vi "libssh2_userauth_authenticated.vi"(8 "error in (no error)":errorcluster, 11 "session":T1) -> (0 "error out":errorcluster, 2 "authenticated":bool)   [LabVIEW 2017, in "libssh2.lvlib"]
doc: "Get a value indicating if a session has been authenticated."
uses:
  libssh2.lvlib
  Session Refnum.ctl
  Not A Session.vi
  <vilib>/Utility/error.llb/Error Cluster From Error Code.vi
  Global Settings.vi
  Read Session Refnum.vi
  <vilib>/Utility/semaphor.llb/Acquire Semaphore.vi
  <vilib>/Utility/semaphor.llb/Release Semaphore.vi
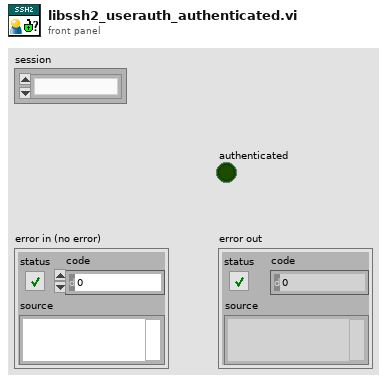
[diagram p1: front panel]
types:
  T1 = typedef "libssh2.lvlib/Session Refnum.ctl" = refnum<k1>
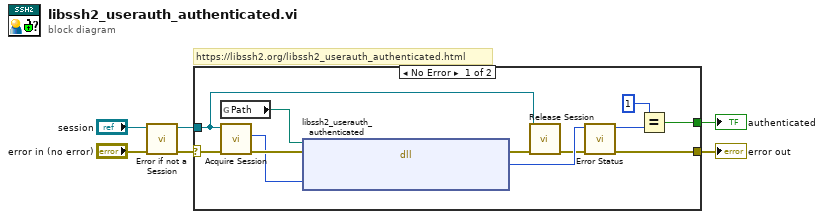
[diagram p0: block diagram]
diagram:
  # "https://libssh2.org/libssh2_userauth_authenticated.html"
  n1 = call "Error if not a Session.vi"("error in (no error)"="error in (no error)", "session"="session") -> ("error out"=w3:errorcluster, "session out"=w1:T1)  [unwired: 8 in]
  n2 = case shown="No Error" w3 {
    selector: w3 -> [w16 w19]
    tunnel: [w13 w19] -> w6
    tunnel: [w10 _] -> w5
    tunnel: w1 -> [w7 _]
    frame No Error {
      n3 = global read "Global Settings.vi" "Path"() -> (w14:path)
      n4 = call "Acquire Session.vi"("error in (no error)"=w16, "session"=w7) -> ("error out"=w18:errorcluster, "LIBSSH2_SESSION*"=w17:u64)  [unwired: 7 in, 1 out]
      n5 = dll-call lib="?" fn="libssh2_userauth_authenticated"(path in=w14, error in=w18, "session"=w17) -> (error out=w15:errorcluster, "return value"=w12:i32)  [unwired: 2 in, 1 out]
      n6 = call "Release Session.vi"("error in (no error)"=w15, "session"=w7) -> ("error out"=w8:errorcluster)  [unwired: 9 in]
      n7 = call "Error Status.vi"("error in (no error)"=w8, "return value"=w12) -> ("error out"=w13:errorcluster, "return value out"=w11:i32)  [unwired: 8 in]
      n8 = Equal?(x=1, y=w11) -> (x = y?=w10:bool)
    }
    frame Error {
    }
  }
  "error out" <- w6
  "authenticated" <- w5
